vi "Invoke Object Method.vi"(8 "error in":errorcluster, 9 "parameters":refnum<k24>[](array[refnum]), 10 "Method Name":string, 11 "Object in":refnum<k24>) -> (0 "error out":errorcluster, 2 "Return Value":refnum<k24>, 3 "Object out":refnum<k24>)   [LabVIEW 2026, in "ToastNotification.lvlib" / "Reflection DotNet.lvlib"]
doc: "Invoke a uniquely named public method on a borrowed .NET object using reflection. Skipped on incoming error. Release acquired Type and MethodInfo even if invocation fails. Return Value is acquired and belongs to the caller; a void method may return null. Does not close Object in or parameter handles. Name-only lookup can fail for overloaded methods."
uses:
  Reflection DotNet.lvlib
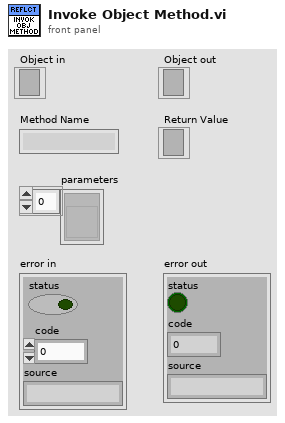
[diagram p1: front panel]
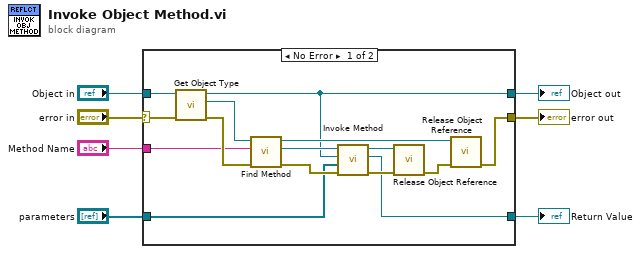
[diagram p0: block diagram]
diagram:
  n1 = case shown="No Error" "error in" {
    selector: "error in" -> [w13 w23]
    tunnel: "Object in" -> [w12 w24]
    tunnel: "Method Name" -> [w14 _]
    tunnel: "parameters" -> [w15 _]
    tunnel: [w8 w24] -> w5
    tunnel: [w19 _] -> w6
    tunnel: [w22 w23] -> w7
    frame No Error {
      n2 = call "Get Object Type.vi"("error in (no error)"=w13, "Object in"=w12) -> ("error out"=w16:errorcluster, "Object Type"=w9:refnum<k24>, "Object out"=w8:refnum<k24>)  [unwired: 7 in]
      n3 = call "Find Method.vi"("error in (no error)"=w16, "Method Name"=w14, "Declaring Type in"=w9) -> ("error out"=w18:errorcluster, "Method Info"=w17:refnum<k24>, "Declaring Type out"=w10:refnum<k24>)  [unwired: 6 in]
      n4 = call "Invoke Method.vi"("error in (no error)"=w18, "parameters"=w15, "Target Object"=w8, "Method Info in"=w17) -> ("error out"=w20:errorcluster, "Return Value"=w19:refnum<k24>, "Method Info out"=w11:refnum<k24>)  [unwired: 5 in]
      n5 = call "Release Object Reference.vi"("error in"=w20, "object"=w11) -> ("error out"=w21:errorcluster)  [unwired: 9 in]
      n6 = call "Release Object Reference.vi"("error in"=w21, "object"=w10) -> ("error out"=w22:errorcluster)  [unwired: 9 in]
    }
    frame Error {
    }
  }
  "Object out" <- w5
  "Return Value" <- w6
  "error out" <- w7
